vi "Open Virtual Folder References.vi"(8 "error in":errorcluster, 10 "lvlib":string, 11 "Project Manager in":refnum<class "Project Manager.lvclass">) -> (0 "error out":errorcluster, 3 "Project Manager out":refnum<class "Project Manager.lvclass">)   [LabVIEW 2026, in "Project Manager.lvclass"]
doc: "Open references to virtual folders in the specified lvlib."
uses:
  Project Manager.lvclass
  Project Manager.lvclass/Project Manager.ctl
  Interfaces/ILogger/ILogger Messages/Log Msg/Log Msg.lvclass/Log Msg.ctl
  <vilib>/ActorFramework/Message Enqueuer/Message Enqueuer.lvclass/Message Enqueuer.ctl
  <vilib>/ActorFramework/Message Enqueuer/Enqueue.vi
  Interfaces/ILogger/ILogger Messages/Log Msg/Log Msg.lvclass
  <vilib>/ActorFramework/Message Priority Queue/Priority Enqueue.vi
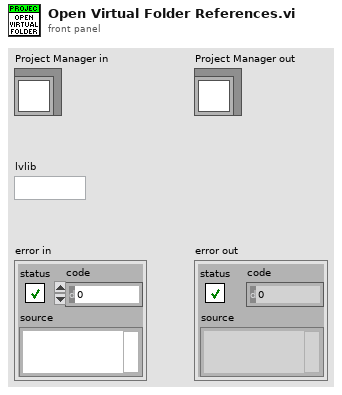
[diagram p1: front panel]
types:
  T1 = typedef "Log Entry--cluster.ctl" = cluster{"Time":timestamp, "Message":string}
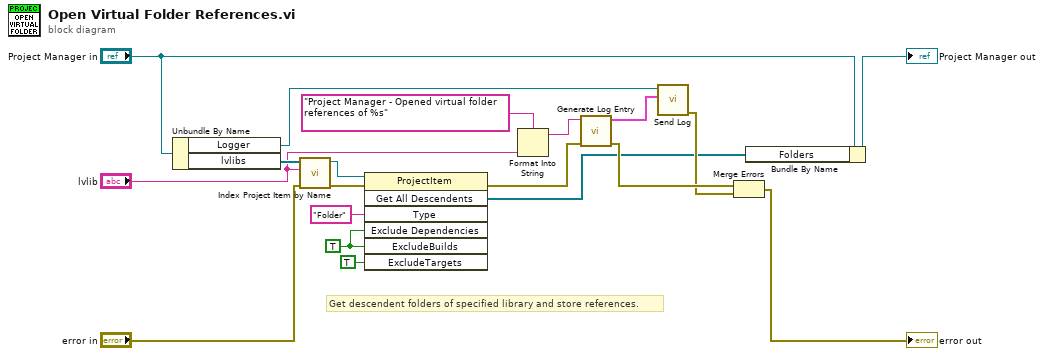
[diagram p0: block diagram]
diagram:
  w11 = TRUE ("ExcludeDependencies")
  # "Get descendent folders of specified library and store references."
  n1 = Unbundle By Name("Project Manager in") -> ("Logger"=w5:refnum<class "Message Enqueuer.lvclass">, "lvlibs"=w12:refnum<vi>[])
  n2 = call "Index Project Item by Name.vi"("error in"="error in", "Name"="lvlib", "Project Items"=w12) -> ("error out"=w18:errorcluster, "Project Item"=w8:refnum<vi>)  [unwired: 7 in]
  n3 = invoke class="ProjectItem" method="Get All Descendents"(reference=w8, error in=w18, "Type"="Folder", "Exclude Dependencies"=w11, "ExcludeBuilds"=w11, "ExcludeTargets"=TRUE) -> (error out=w17:errorcluster, "All Descendents"=w6:refnum<vi>[])  [unwired: 1 in, 5 out]
  n4 = Format Into String(format string="Project Manager - Opened virtual folder references of %s" ("Message"), "lvlib") -> (resulting string=w2:string)  [unwired: 2 in, 1 out]
  n5 = call "Generate Log Entry.vi"("error in"=w17, "Message"=w2) -> ("error out"=w16:errorcluster, "Log Entry"=w1:T1)  [unwired: 8 in]
  n6 = call "Send Log.vi"("Log Entry"=w1, "Message Enqueuer"=w5) -> ("error out"=w14:errorcluster)  [unwired: 8 in, 1 out]
  n7 = Merge Errors(w16, w14) -> (→"error out":errorcluster)
  n8 = Bundle By Name(cluster="Project Manager in", "Folders"=w6) -> (→"Project Manager out":refnum<class "Project Manager.lvclass">)
